vi "example 4b - string.vi"() -> ()   [LabVIEW 2020]
uses:
  ui-testing/ui-testing.lvlib
panel:
  in  "Tree":string[](tree)
  in  "String":string
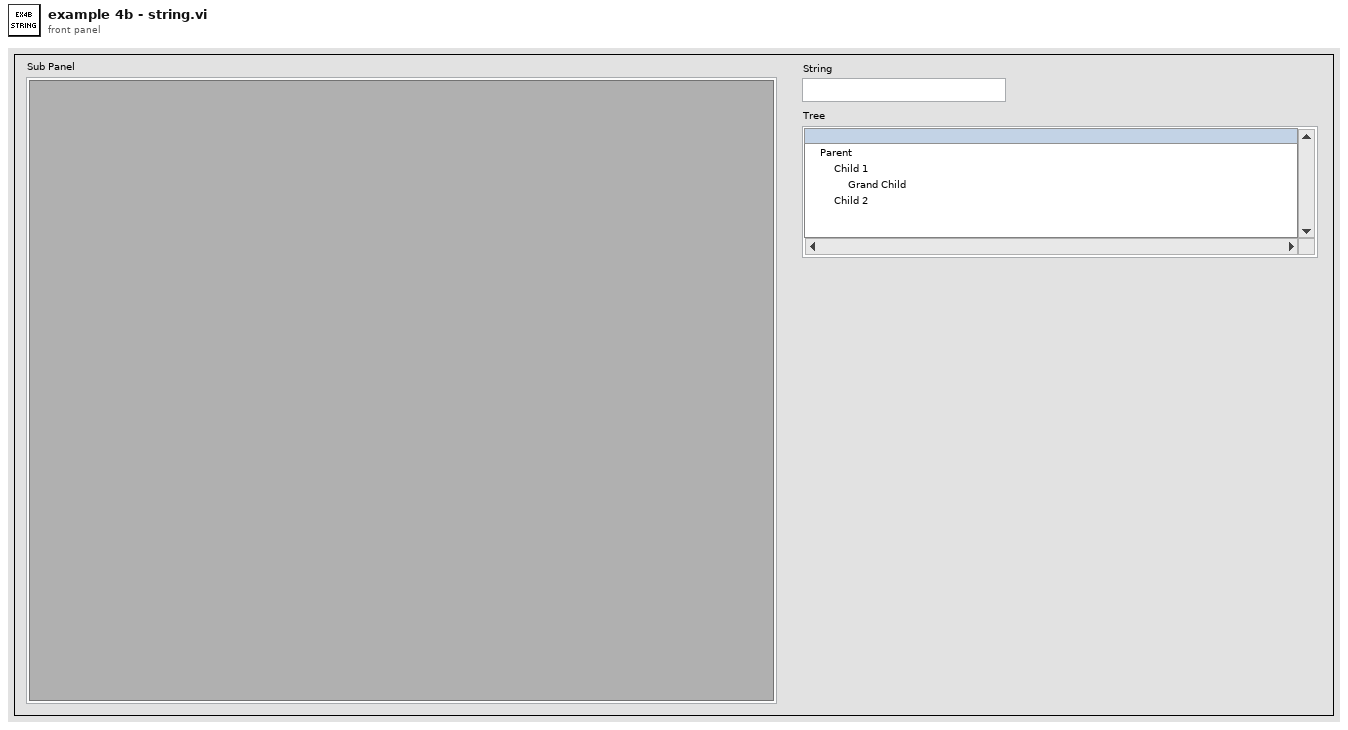
[diagram p1: front panel]
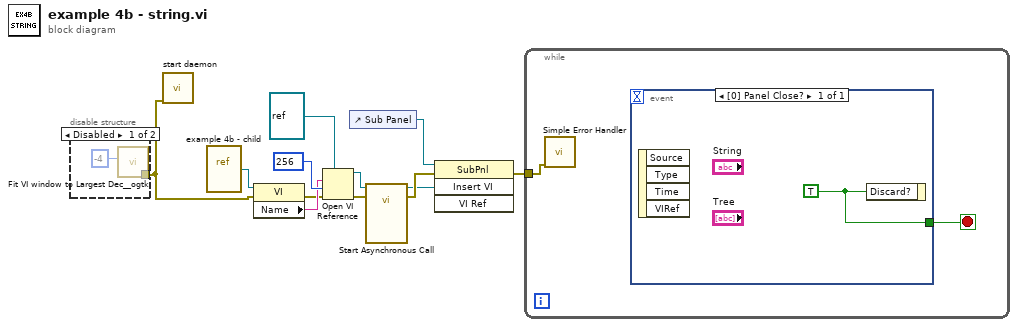
[diagram p0: block diagram]
diagram:
  n1 = disable-structure shown="Disabled" {
    disable-tunnel: [w13 _] -> w1
    frame Disabled {
      n2 = call <userlib>:"Fit VI window to Largest Dec__ogtk.vi"("border spacing (2 px)"=-4) -> ("error out"=w13:errorcluster)  [unwired: 5 in, 1 out]
    }
    frame Enabled {
    }
  }
  n3 = call "start daemon.vi"("error in (no error)"=w1) -> ()  [unwired: 10 in, 1 out]
  n4 = vi-ref "example 4b - child.vi"() -> (w8:refnum<vi>)
  n5 = property class="VI"(reference=w8, error in=w1) -> (error out=w6:errorcluster, "Name"=w7:string)  [unwired: 1 out]
  n6 = Open VI Reference(type specifier VI Refnum (for type only)=refnum<vi> refnum, vi path=w7, options=256 ("call and forget"), error in (no error)=w6) -> (vi reference=w10:refnum<vi>, error out=w9:errorcluster)  [unwired: 2 in]
  n7 = control-ref of="Sub Panel"() -> (w2:refnum<vi>)
  n8 = call-by-ref "Start Asynchronous Call"(reference=w10, error in=w9) -> (reference out=w4:refnum<vi>, error out=w5:errorcluster)  [unwired: 12 in]
  n9 = invoke on="Invoke Node" class="SubPnl" method="Insert VI"(reference=w2, error in=w5, "VI Ref"=w4) -> (error out=w3:errorcluster)  [unwired: 1 in, 3 out]
  n10 = while {
    tunnel: w3 -> [w15]
    stop <- w16 stop-if-true
    n11 = call <vilib>:"Simple Error Handler.vi"("error in (no error)"=w15) -> ()  [unwired: 4 in, 5 out]
    n12 = event shown="[0] Panel Close?" {
      selector: _ -> [_]
      dyn-events: _ -> [_]
      timeout: _ -> [_]
      tunnel: [w17] -> w16
      event Panel Close? {
        w17 = TRUE
        n13 = event-data() -> ()  [unwired: 1 in, 4 out]
        n14 = event-data("Discard?"=w17) -> ()  [unwired: 1 in, 1 out]
      }
    }
  }
